vi "Element Type.vi"(11 "NumericCommandButton in":refnum<class "NumericCommandButton.lvclass">) -> (2 "Element Type":string)   [LabVIEW 2025, in "VolatusGUIElements.lvlib" / "NumericCommandButton.lvclass"]
uses:
  NumericCommandButton.lvclass
  NumericCommandButton.lvclass/NumericCommandButton.ctl
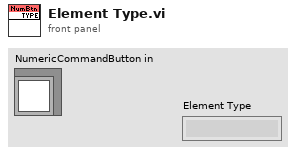
[diagram p1: front panel]
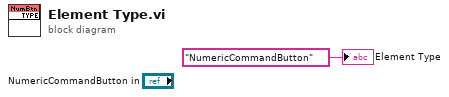
[diagram p0: block diagram]
diagram:
  "Element Type" <- "NumericCommandButton" ("Element Type")
